vi "RDC-permittivity-Bilinear_format.vi"(7 "basic data(open, short, water)":T1[](array[typedef]), 11 "Common Format":T1) -> (3 "Common Format out":T1)   [LabVIEW 2020, in "RDC-Reflection_Data_Computation.lvlib"]
doc: "Prepares the basic data (open, short, water) with RDC-add_ideal_perm and computes the permittivity of a Common Format cluster with RDC-permittivity-Bilinear."
uses:
  RDC-Reflection_Data_Computation.lvlib
  Reflector/RFH-common_data_format.ctl
  Reflector/RFH-Reflection_File_Handler.lvlib
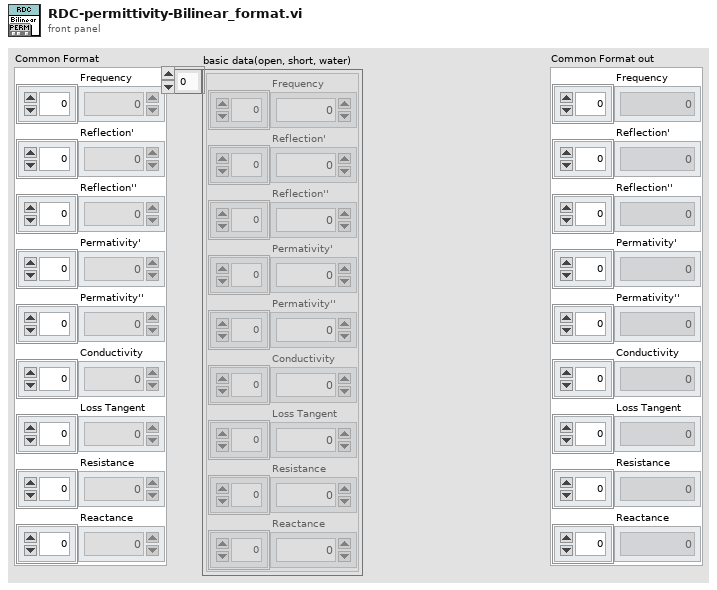
[diagram p1: front panel]
types:
  T1 = typedef "RFH-Reflection_File_Handler.lvlib/RFH-common_data_format.ctl" = cluster{"Frequency":dbl[], "Reflection'":dbl[], "Reflection''":dbl[], "Permativity'":dbl[], "Permativity''":dbl[], "Conductivity":dbl[], "Loss Tangent":dbl[], "Resistance":dbl[], "Reactance":dbl[]}
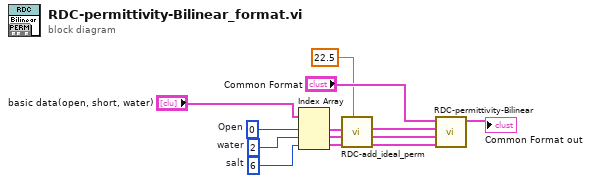
[diagram p0: block diagram]
diagram:
  w10 = 6  # salt
  w11 = 2  # water
  w12 = 0  # Open
  n1 = Index Array(array="basic data(open, short, water)", index #1=w12, index #2=w11, index #3=w10) -> (element #1=w7:T1, element #2=w5:T1, element #3=w4:T1)
  n2 = call "RDC-add_ideal_perm.vi"("water Temp (25C) [10-40C]"=22.5, "Salt Water"=w4, "DI-Water"=w5, "Open/Air"=w7) -> ("Salt Water out"=w1:T1, "DI-Water  out"=w2:T1, "Open/Air out"=w3:T1)  [unwired: 5 in]
  n3 = call "RDC-permittivity-Bilinear.vi"("Salt Water"=w1, "DI-Water"=w2, "Open/Air"=w3, "Common Format"="Common Format") -> ("Common Format out"=→"Common Format out":T1)  [unwired: 7 in]
